vi "Update Library Icon.vi"(8 "error in (no error)":errorcluster, 11 "Mock Class Generator In":refnum<class "Mock Class Generator.lvclass">) -> (0 "error out":errorcluster, 3 "Mock Class Generator Out":refnum<class "Mock Class Generator.lvclass">)   [LabVIEW 2020, in "Mock Class Generator.lvclass"]
uses:
  Mock Class Generator.lvclass
  <vilib>/LabVIEW Icon API/lv_icon/Classes/Icon/Icon.lvclass
  <vilib>/LabVIEW Icon API/API_Rectangle Dimension.ctl
  <vilib>/LabVIEW Icon API/API_Text.ctl
  <vilib>/LabVIEW Icon API/API_Test Settings.ctl
  <vilib>/LabVIEW Icon API/lv_icon/Controls/Alignment.ctl
  <vilib>/LabVIEW Icon API/API_Text Colors.ctl
  <vilib>/LabVIEW Icon API/API_Rectangle Colors.ctl
  Mock Class Generator.lvclass/Mock Class Generator.ctl
  <vilib>/LabVIEW Icon API/LabVIEW Icon API.lvlib
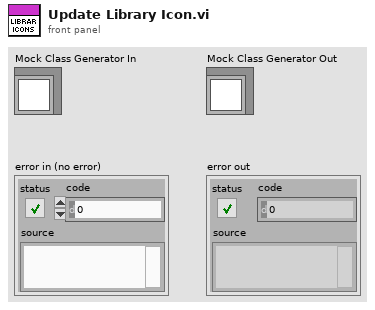
[diagram p1: front panel]
types:
  T1 = typedef "LabVIEW Icon API.lvlib/API_Rectangle Colors.ctl" = cluster{"Border":u32, "Background":u32}
  T2 = typedef "LabVIEW Icon API.lvlib/API_Test Settings.ctl" = cluster{"Font":string, "Alignment":T3, "Size":u8, "Center text":bool, "Capitalize text":bool, "Text color":T4}
  T3 = typedef "Alignment.ctl" = u16
  T4 = typedef "LabVIEW Icon API.lvlib/API_Text Colors.ctl" = cluster{"Line 1 color":u32, "Line 2 color":u32, "Line 3 color":u32, "Line 4 color":u32}
  T5 = typedef "LabVIEW Icon API.lvlib/API_Text.ctl" = cluster{"Line 1 text":string, "Line 2 text":string, "Line 3 text":string, "Line 4 text":string}
  T6 = typedef "LabVIEW Icon API.lvlib/API_Rectangle Dimension.ctl" = cluster{"Width":i16, "Height":i16}
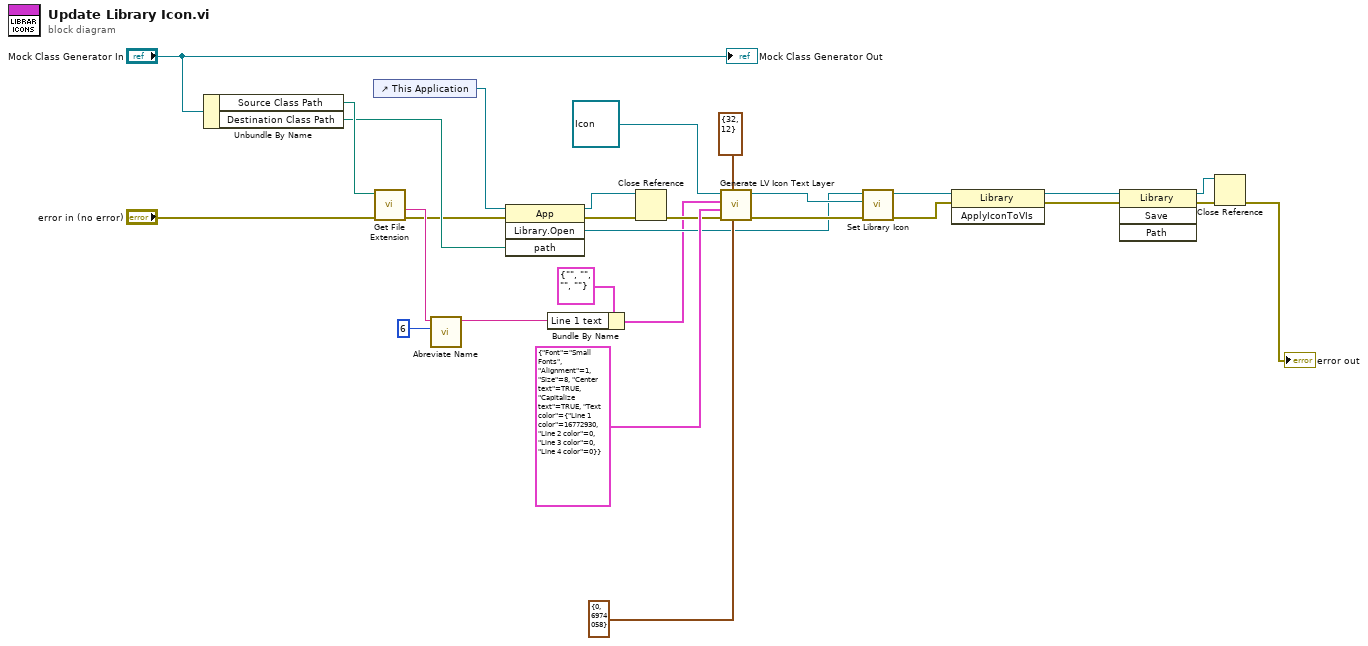
[diagram p0: block diagram]
diagram:
  n1 = Unbundle By Name("Mock Class Generator In") -> ("Source Class Path"=w22:path, "Destination Class Path"=w16:path)
  n2 = control-ref of="This Application"() -> (w17:refnum<vi>)
  n3 = call <vilib>:"Get File Extension.vi"("error in (no error)"="error in (no error)", "file"=w22) -> ("error out"=w12:errorcluster, "filename without extension"=w21:string)  [unwired: 5 in, 3 out]
  n4 = call "Abreviate Name.vi"("Max Length"=6, "Long Name in"=w21) -> ("Long Name out"=w18:string)  [unwired: 9 in]
  n5 = invoke class="App" method="Library.Open"(reference=w17, error in=w12, "path"=w16) -> (reference out=w2:refnum<vi>, error out=w11:errorcluster, "Open Library"=w10:refnum<vi>)  [unwired: 1 in, 1 out]
  n6 = Bundle By Name(cluster=T5 {"Line 1 text"="", "Line 2 text"="", "Line 3 text"="", "Line 4 text"=""} ("Text"), "Line 1 text"=w18) -> (w1:T5)
  n7 = Close Reference(reference=w2, error in (no error)=w11) -> (error out=w3:errorcluster)
  n8 = call <vilib>:"Generate LV Icon Text Layer.vi"("Rectangle colors (black, white)"=T1 {"Border"=0, "Background"=6974058}, "Rectangle dimension (32,32)"=T6 {"Width"=32, "Height"=12}, "error in (no error)"=w3, "Text settings"=T2 {"Font"="Small Fonts", "Alignment"=1, "Size"=8, "Center text"=TRUE, "Capitalize text"=TRUE, "Text color"={"Line 1 color"=16772930, "Line 2 color"=0, "Line 3 color"=0, "Line 4 color"=0}}, "Text"=w1, "Icon in"=refnum<class "Icon.lvclass"> refnum ("Icon.lvclass in")) -> ("error out"=w14:errorcluster, "Icon out"=w20:refnum<class "Icon.lvclass">)  [unwired: 4 in]
  n9 = call <vilib>:"Set Library Icon.vi"("error in (no error)"=w14, "Icon"=w20, "Library Refnum in"=w10) -> ("error out"=w13:errorcluster, "Library Refnum out"=w8:refnum<vi>)  [unwired: 7 in]
  n10 = invoke class="Library" method="ApplyIconToVIs"(reference=w8, error in=w13) -> (reference out=w5:refnum<vi>, error out=w9:errorcluster)  [unwired: 1 in, 1 out]
  n11 = invoke class="Library" method="Save"(reference=w5, error in=w9) -> (reference out=w4:refnum<vi>, error out=w7:errorcluster)  [unwired: 2 in, 2 out]
  n12 = Close Reference(reference=w4, error in (no error)=w7) -> (error out=→"error out":errorcluster)
  "Mock Class Generator Out" <- "Mock Class Generator In"
